vi "MQTT Reason HANDLER.vi"(5 "MessageType":T1, 7 "Reason Code":u8, 11 "error in (no error)":errorcluster) -> (15 "error out":errorcluster)   [LabVIEW 2019, in "KoRE-MQTT.lvlib"]
doc: "Copyright (c) 2025 KoRElibs.com\nSPDX-License-Identifier: EUPL-1.2\n\nThis VI is licensed under the European Union Public License (EUPL) Version 1.2. You may use this VI unmodified in proprietary works. If you distribute a modified version of this file, the modified file must be released under the EUPL-1.2. Full license: https://joinup.ec.europa.eu/asset/eupl/eupl/1.2/"
uses:
  KoRE-MQTT.lvlib
  TypeDefs/MQTT Packet - Type.ctl
panel:
  out "DEBUG":string[][](array[string])
  out "DEBUG - Reason":string
  out "DEBUG - Acion":string
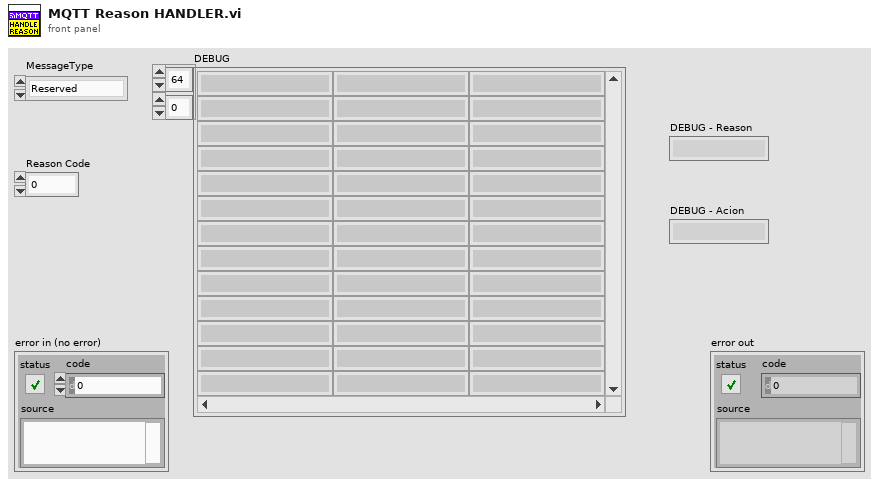
[diagram p1: front panel]
types:
  T1 = typedef "KoRE-MQTT.lvlib/MQTT Packet - Type.ctl" = enum32{"Reserved", "CONNECT", "CONNACK", "PUBLISH", "PUBACK", "PUBREC", "PUBREL", "PUBCOMP", "SUBSCRIBE", "SUBACK", "UNSUBSCRIBE", "UNSUBACK", "PINGREQ", "PINGRESP", "DISCONNECT", "AUTH"}
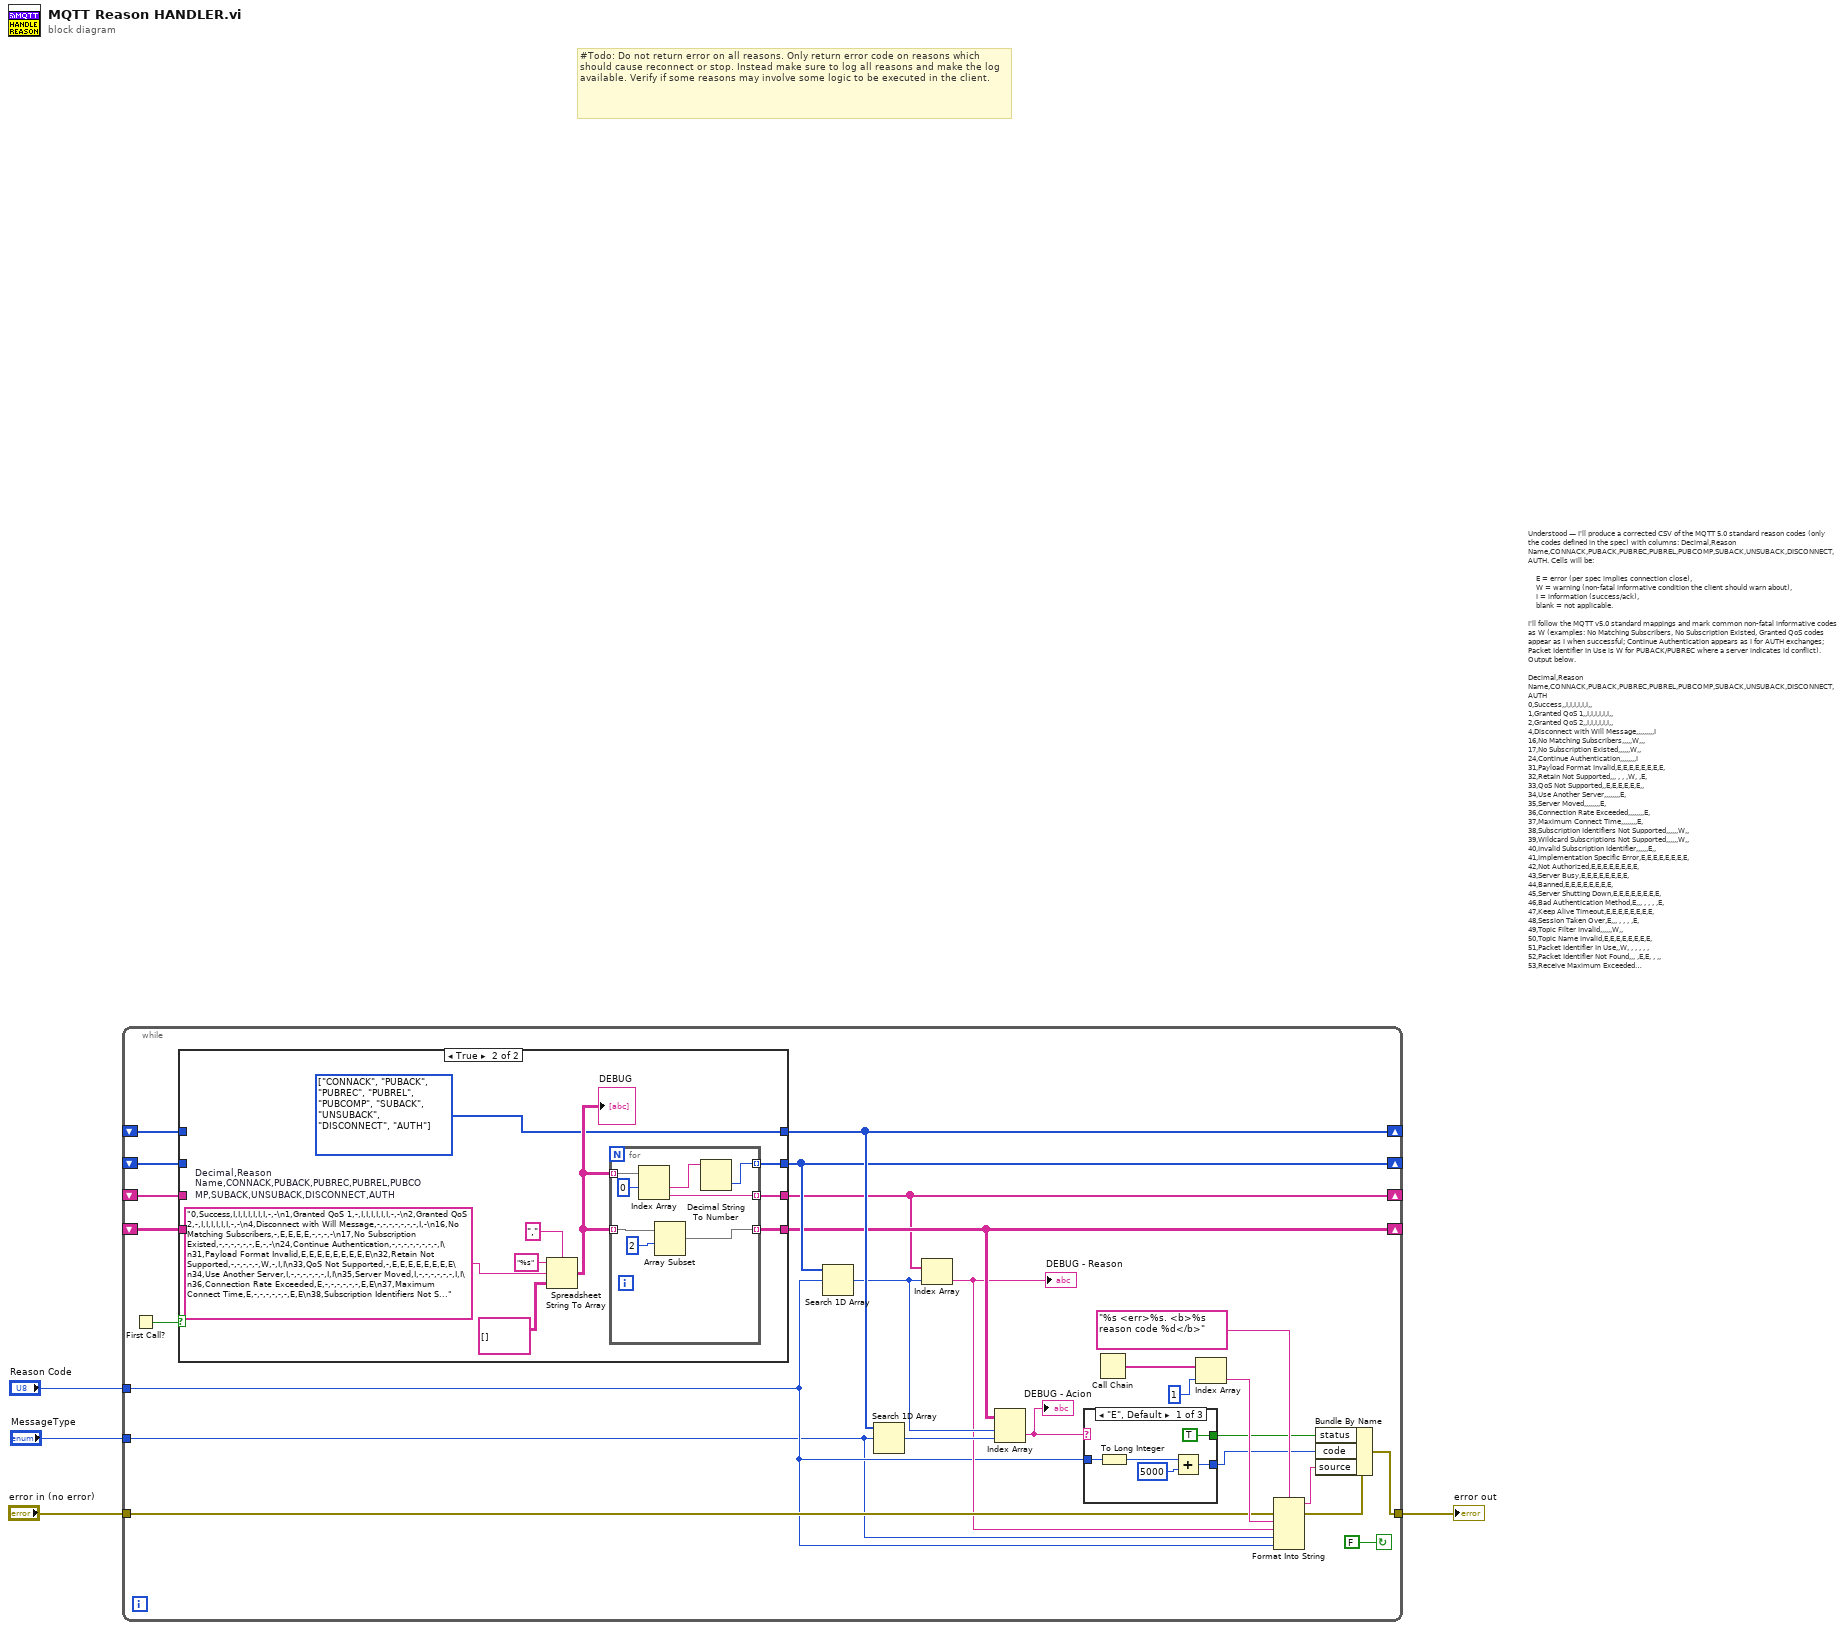
[diagram p0: block diagram]
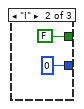
[diagram p3: hidden frame]
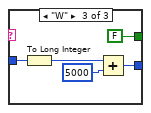
[diagram p4: hidden frame]
diagram:
  # "Understood — I'll produce a corrected CSV of the MQTT 5.0 standard reason codes (only the codes defined in the spec) with columns: Decimal,Reason Name,CONNACK,PUBACK,PUBREC,PUBREL,PUBCOMP,SUBACK,UNSUBACK,DISCONNECT,AUTH. Cells will be:\n\n    E = error (per spec implies connection close),\n    W = warning (non-fatal informative condition the client should warn about),\n    I = information (success/ack),\n    blank = not applicable.\n\nI'll follow the MQTT v5.0 standard mappings and mark common non-fatal informative codes as W (examples: No Matching Subscribers, No Subscription Existed, Granted QoS codes appear as I when successful; Continue Authentication appears as I for AUTH exchanges; Packet Identifier In Use is W for PUBACK/PUBREC where a server indicates id conflict). Output below.\n\nDecimal,Reason Name,CONNACK,PUBACK,PUBREC,PUBREL,PUBCOMP,SUBACK,UNSUBACK,DISCONNECT,AUTH\n0,Success,,I,I,I,I,I,I,,\n1,Granted QoS 1,,I,I,I,I,I,I,,\n2,Granted QoS 2,,I,I,I,I,I,I,,\n4,Disconnect with Will Message,,,,,,,,,I\n16,No Matching Subscribers,,,,,W,,,\n17,No Subscription Existed,,,,,,W,,\n24,Continue Authentication,,,,,,,,I\n31,Payload Format Invalid,E,E,E,E,E,E,E,E,\n32,Retain Not Supported,,, , , ,W, ,E,\n33,QoS Not Supported,,E,E,E,E,E,E,,\n34,Use Another Server,,,,,,,,E,\n35,Server Moved,,,,,,,,E,\n36,Connection Rate Exceeded,,,,,,,,E,\n37,Maximum Connect Time,,,,,,,,E,\n38,Subscription Identifiers Not Supported,,,,,,W,,\n39,Wildcard Subscriptions Not Supported,,,,,,W,,\n40,Invalid Subscription Identifier,,,,,,E,,\n41,Implementation Specific Error,E,E,E,E,E,E,E,E,\n42,Not Authorized,E,E,E,E,E,E,E,E,\n43,Server Busy,E,E,E,E,E,E,E,E,\n44,Banned,E,E,E,E,E,E,E,E,\n45,Server Shutting Down,E,E,E,E,E,E,E,E,\n46,Bad Authentication Method,E,,, , , , ,E,\n47,Keep Alive Timeout,E,E,E,E,E,E,E,E,\n48,Session Taken Over,E,,, , , , ,E,\n49,Topic Filter Invalid,,,,,,W,,\n50,Topic Name Invalid,E,E,E,E,E,E,E,E,\n51,Packet Identifier In Use,,W, , , , , ,\n52,Packet Identifier Not Found,,, ,E,E, , ,,\n53,Receive Maximum Exceeded,,W,W,W,W, , ,E,\n54,Topic Alias Invalid,E,E,E,E,E,E,E,E,\n55,Packet Too Large,E,E,E,E,E,E,E,E,\n56,Message Rate Too High,,W,W,W,W, , ,E,\n57,Quota Exceeded,E,E,E,E,E,E,E,E,\n58,Administrative Action,E,E,E,E,E,E,E,E,\n128,Unspecified Error,E,E,E,E,E,E,E,E,\n129,Malformed Packet,E,E,E,E,E,E,E,E,\n130,Protocol Error,E,E,E,E,E,E,E,E,\n131,Implementation Specific Error,E,E,E,E,E,E,E,E,\n132,Not Authorized,E,E,E,E,E,E,E,E,\n133,Server Busy,E,E,E,E,E,E,E,E,\n134,Server Shutting Down,E,E,E,E,E,E,E,E,\n135,Bad Authentication Method,E,,, , , , ,E,\n136,Keep Alive Timeout,E,E,E,E,E,E,E,E,\n137,Session Taken Over,E,,, , , , ,E,\n138,Topic Filter Invalid,,,,,,W,,\n139,Topic Name Invalid,E,E,E,E,E,E,E,E,\n140,Receive Maximum Exceeded,,W,W,W,W, , ,E,\n141,Topic Alias Invalid,E,E,E,E,E,E,E,E,\n142,Packet Too Large,E,E,E,E,E,E,E,E,\n143,Message Rate Too High,E,E,E,E,E,E,E,E,\n144,Quota Exceeded,E,E,E,E,E,E,E,E,\n145,Administrative Action,E,E,E,E,E,E,E,E,\n146,Packet Identifier Not Found,,, ,E,E, , ,,\n147,Payload Format Invalid,E,E,E,E,E,E,E,E,\n148,Retention Not Supported,,,,,,W,,\n149,QoS Not Supported,E,E,E,E,E,E,E,E,\n150,Use Another Server,,,,,,,,E,\n151,Server Moved,,,,,,,,E,\n152,Shared Subscriptions Not Supported,,,,,,W,,\n153,Connection Rate Exceeded,,,,,,,,E,\n154,Maximum Connect Time,,,,,,,,E,\n155,Subscription Identifiers Not Supported,,,,,,W,,\n156,Wildcard Subscriptions Not Supported,,,,,,W,,\n157,Invalid Authorization Credentials,E,,, , , , ,E,\n158,Retain Not Supported,,,,,,W,,\n159,QoS Not Supported,E,E,E,E,E,E,E,E,\n160,Use Another Server,,,,,,,,E,\n161,Server Moved,,,,,,,,E,\n162,Shared Subscriptions Not Supported,,,,,,W,,\n163,Connection Rate Exceeded,,,,,,,,E,\n164,Maximum Connect Time,,,,,,,,E,\n165,Subscription Identifiers Not Supported,,,,,,W,,\n166,Wildcard Subscriptions Not Supported,,,,,,W,,\n167,Invalid Authorization Credentials,E,,, , , , ,E"
  # "#Todo: Do not return error on all reasons. Only return error code on reasons which should cause reconnect or stop. Instead make sure to log all reasons and make the log available. Verify if some reasons may involve some logic to be executed in the client."
  n1 = while {
    shift-right: [w24] -> _
    shift-left: _ -> [w29]
    shift-right: [w23] -> _
    shift-left: _ -> [w28]
    shift-right: [w21] -> _
    shift-left: _ -> [w27]
    shift-right: [w25] -> _
    shift-left: _ -> [w26]
    tunnel: [w14] -> w4
    tunnel: "error in (no error)" -> [w13]
    tunnel: "Reason Code" -> [w6]
    tunnel: "MessageType" -> [w5]
    stop <- FALSE continue-if-true
    n2 = First Call?() -> (First Call?: T/F=w30:bool)
    n3 = case shown="True" w30 {
      tunnel: [w34 w39] -> w24
      tunnel: w29 -> [w34 _]
      tunnel: [w31 w36] -> w23
      tunnel: w28 -> [w31 _]
      tunnel: [w32 w37] -> w21
      tunnel: w27 -> [w32 _]
      tunnel: [w33 w35] -> w25
      tunnel: w26 -> [w33 _]
      frame False {
      }
      frame True {
        w35 = T1[] [enum."CONNACK", enum."PUBACK", enum."PUBREC", enum."PUBREL", enum."PUBCOMP", enum."SUBACK", enum."UNSUBACK", enum."DISCONNECT", enum."AUTH"] items=["Reserved", "CONNECT", "CONNACK", "PUBLISH", "PUBACK", "PUBREC", "PUBREL", "PUBCOMP", "SUBSCRIBE", "SUBACK", "UNSUBSCRIBE", "UNSUBACK", "PINGREQ", "PINGRESP", "DISCONNECT", "AUTH"]
        w43 = "0,Success,I,I,I,I,I,I,I,-,-\n1,Granted QoS 1,-,I,I,I,I,I,I,-,-\n2,Granted QoS 2,-,I,I,I,I,I,I,-,-\n4,Disconnect with Will Message,-,-,-,-,-,-,-,I,-\n16,No Matching Subscribers,-,E,E,E,E,-,-,-,-\n17,No Subscription Existed,-,-,-,-,-,-,E,-,-\n24,Continue Authentication,-,-,-,-,-,-,-,-,I\n31,Payload Format Invalid,E,E,E,E,E,E,E,E,E\n32,Retain Not Supported,-,-,-,-,-,W,-,I,I\n33,QoS Not Supported,-,E,E,E,E,E,E,E,E\n34,Use Another Server,I,-,-,-,-,-,-,I,I\n35,Server Moved,I,-,-,-,-,-,-,I,I\n36,Connection Rate Exceeded,E,-,-,-,-,-,-,E,E\n37,Maximum Connect Time,E,-,-,-,-,-,-,E,E\n38,Subscription Identifiers Not Supported,-,-,-,-,-,W,W,-,-\n39,Wildcard Subscriptions Not Supported,-,-,-,-,-,W,W,-,-\n40,Invalid Subscription Identifier,-,-,-,-,-,E,-,-,-\n41,Implementation Specific Error,E,E,E,E,E,E,E,E,E\n42,Not Authorized,E,E,E,E,E,E,E,E,E\n43,Server Busy,E,E,E,E,E,E,E,E,E\n44,Banned,E,E,E,E,E,E,E,E,E\n45,Server Shutting Down,E,E,E,E,E,E,E,E,E\n46,Bad Authentication Method,E,-,-,-,-,-,-,I,I\n47,Keep Alive Timeout,E,E,E,E,E,E,E,E,E\n48,Session Taken Over,E,-,-,-,-,-,-,I,I\n49,Topic Filter Invalid,-,-,-,-,-,W,W,-,-\n50,Topic Name Invalid,E,E,E,E,E,E,E,E,E\n51,Packet Identifier In Use,-,W,W,W,W,W,W,-,-\n52,Packet Identifier Not Found,-,-,E,E,-,-,-,-,-\n53,Receive Maximum Exceeded,-,W,W,W,W,W,W,E,E\n54,Topic Alias Invalid,E,E,E,E,E,E,E,E,E\n55,Packet Too Large,E,E,E,E,E,E,E,E,E\n56,Message Rate Too High,-,W,W,W,W,W,W,E,E\n57,Quota Exceeded,E,E,E,E,E,E,E,E,E\n58,Administrative Action,E,E,E,E,E,E,E,E,E\n128,Unspecified Error,E,E,E,E,E,E,E,E,E\n129,Malformed Packet,E,E,E,E,E,E,E,E,E\n130,Protocol Error,E,E,E,E,E,E,E,E,E\n131,Implementation Specific Error,E,E,E,E,E,E,E,E,E\n132,Not Authorized,E,E,E,E,E,E,E,E,E\n133,Server Busy,E,E,E,E,E,E,E,E,E\n134,Server Shutting Down,E,E,E,E,E,E,E,E,E\n135,Bad Authentication Method,E,-,-,-,-,-,-,I,I\n136,Keep Alive Timeout,E,E,E,E,E,E,E,E,E\n137,Session Taken Over,E,-,-,-,-,-,-,I,I\n138,Topic Filter Invalid,-,-,-,-,-,W,W,-,-\n139,Topic Name Invalid,E,E,E,E,E,E,E,E,E\n140,Receive Maximum Exceeded,-,W,W,W,W,W,W,E,E\n141,Topic Alias Invalid,E,E,E,E,E,E,E,E,E\n142,Packet Too Large,E,E,E,E,E,E,E,E,E\n143,Message Rate Too High,E,E,E,E,E,E,E,E,E\n144,Quota Exceeded,E,E,E,E,E,E,E,E,E\n145,Administrative Action,E,E,E,E,E,E,E,E,E\n146,Packet Identifier Not Found,-,-,W,W,-,-,-,-,-\n147,Payload Format Invalid,E,E,E,E,E,E,E,E,E\n148,Retention Not Supported,-,-,-,-,-,W,W,-,-\n149,QoS Not Supported,-,E,E,E,E,E,E,E,E\n150,Use Another Server,I,-,-,-,-,-,-,I,I\n151,Server Moved,I,-,-,-,-,-,-,I,I\n152,Shared Subscriptions Not Supported,-,-,-,-,-,W,W,-,-\n153,Connection Rate Exceeded,E,-,-,-,-,-,-,E,E\n154,Maximum Connect Time,E,-,-,-,-,-,-,E,E\n155,Subscription Identifiers Not Supported,-,-,-,-,-,W,W,-,-\n156,Wildcard Subscriptions Not Supported,-,-,-,-,-,W,W,-,-\n157,Invalid Authorization Credentials,E,-,-,-,-,-,-,I,I\n158,Retain Not Supported,-,-,-,-,-,W,W,I,I\n159,QoS Not Supported,E,E,E,E,E,E,E,E,E\n160,Use Another Server,I,-,-,-,-,-,-,I,I\n161,Server Moved,I,-,-,-,-,-,-,I,I\n162,Shared Subscriptions Not Supported,-,-,-,-,-,W,W,-,-\n163,Connection Rate Exceeded,E,-,-,-,-,-,-,E,E\n164,Maximum Connect Time,E,-,-,-,-,-,-,E,E\n165,Subscription Identifiers Not Supported,-,-,-,-,-,W,W,-,-\n166,Wildcard Subscriptions Not Supported,-,-,-,-,-,W,W,-,-\n167,Invalid Authorization Credentials,E,-,-,-,-,-,-,I,I"  # Decimal,Reason Name,CONNACK,PUBACK,PUBREC,PUBREL,PUBCOMP,SUBACK,UNSUBACK,DISCONNECT,AUTH
        n4 = Spreadsheet String To Array(delimiter (Tab)=",", format string="%s", spreadsheet string=w43, array type (2D Dbl)=string[][] []) -> (array=w38:string[][])
        "DEBUG" <- w38
        n5 = for {
          tunnel: w38 -> [w51] mode=indexing
          tunnel: [w48] -> w39 mode=indexing
          tunnel: w38 -> [w45] mode=indexing
          tunnel: [w47] -> w37 mode=indexing
          tunnel: [w44] -> w36 mode=indexing
          n6 = Index Array(array=w51, index #1=0 ("index")) -> (element #1=w49:string, element #2=w47:string)  [unwired: 1 in]
          n7 = Array Subset(array=w45, index=2) -> (w44:string[])  [unwired: 1 in]
          n8 = Decimal String To Number(string=w49) -> (number=w48:i32)  [unwired: 2 in, 1 out]
        }
      }
    }
    n9 = Search 1D Array(1D array=w24, element=w6) -> (index of element=w20:i32)  [unwired: 1 in]
    n10 = Search 1D Array(1D array=w25, element=w5) -> (index of element=w22:i32)  [unwired: 1 in]
    n11 = Index Array(array=w21, index=w20) -> (element=w11:string)
    "DEBUG - Reason" <- w11
    n12 = Index Array(array=w23, index (row)=w20, index (col)=w22) -> (element=w10:string)
    "DEBUG - Acion" <- w10
    n13 = case shown="\"E\", Default" w10 {
      tunnel: [TRUE ("status") FALSE ("status") FALSE ("status")] -> w15
      tunnel: [w53 0 w60] -> w8
      tunnel: w6 -> [w52 _ w59]
      frame "E", Default {
        n14 = To Long Integer(number=w52) -> (32bit integer=w55:i32)
        n15 = Add(x=w55, y=5000 ("code")) -> (x+y=w53:i32)
      }
      frame "I" {
      }
      frame "W" {
        n16 = To Long Integer(number=w59) -> (32bit integer=w62:i32)
        n17 = Add(x=w62, y=5000 ("code")) -> (x+y=w60:i32)
      }
    }
    n18 = Call Chain() -> (call chain=w19:string[])
    n19 = Index Array(array=w19, index=1) -> (element=w18:string)
    n20 = Format Into String(format string="%s <err>%s. <b>%s reason code %d</b>", error in=w13, w18, w11, w5, w6) -> (resulting string=w7:string, error out=w12:errorcluster)  [unwired: 1 in]
    n21 = Bundle By Name(cluster=w12, "status"=w15, "code"=w8, "source"=w7) -> (w14:errorcluster)
  }
  "error out" <- w4
